vi "Format Double Numeric.vi"(1 "value":dbl) -> (0 "String":string)   [LabVIEW 2020, in "Astemes_CSVReportPlugin.lvlib" / "TestStand Result Handler.lvclass"]
uses:
  TestStand Result Handler.lvclass
  TestStand Result Handler.lvclass/TestStand Result Handler.ctl
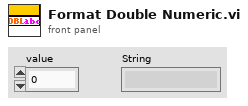
[diagram p1: front panel]
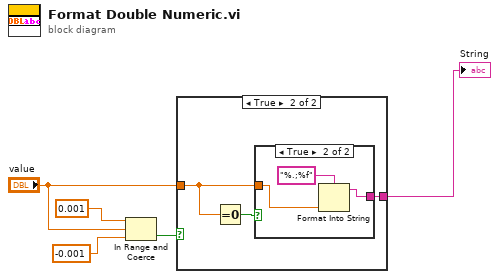
[diagram p0: block diagram]
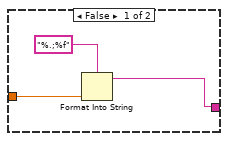
[diagram p2: hidden frame]
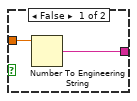
[diagram p3: hidden frame]
diagram:
  n1 = In Range and Coerce(upper limit=0.001 ("y"), x="value", lower limit=-0.001 ("y")) -> (In Range?=w1:bool)  [unwired: 1 out]
  n2 = case shown="True" w1 {
    tunnel: "value" -> [w7 w10]
    tunnel: [w6 w11] -> w5
    frame False {
      n3 = Format Into String(format string="%.;%f", w7) -> (resulting string=w6:string)  [unwired: 2 in, 1 out]
    }
    frame True {
      n4 = Equal To 0?(x=w10) -> (x = 0?=w9:bool)
      n5 = case shown="True" w9 {
        tunnel: [w13 w14] -> w11
        tunnel: w10 -> [w12 w15]
        frame False {
          n6 = Number To Engineering String(4:w12) -> (0:w13:string)  [unwired: 3 in]
        }
        frame True {
          n7 = Format Into String(format string="%.;%f", w15) -> (resulting string=w14:string)  [unwired: 2 in, 1 out]
        }
      }
    }
  }
  "String" <- w5
